vi "Acquire Data.vi"(7 "user event":T2, 8 "error in (no error)":errorcluster, 9 "UI Refs":T1, 10 "Waveforms":waveform(dbl)[](array[waveform]), 11 "XY Plotter":refnum<class "XY Plotter.lvclass">) -> (0 "error out":errorcluster, 3 "XY Plotter out":refnum<class "XY Plotter.lvclass">)   [LabVIEW 2025, in "XY Plotter.lvlib" / "XY Plotter.lvclass"]
uses:
  XY Plotter.lvclass
  Users/Public/Documents/Sandia National Labs/TSS Plugin/CEF.lvlibp/Node/UserEventRef.ctl
  XY Plotter configuration/XY Plotter configuration.lvclass
  XY Plotter configuration/XY Plotter configuration.lvclass/XY Plotter configuration.ctl
  41d9ed76-e5e6-4aa3-be95-e74946f1bf3d.vi
  XY Plotter configuration/Read XY Plotter.vi
  Users/Public/Documents/Sandia National Labs/TSS Plugin/CEF.lvlibp/serializable configuration/CEF_serializable configuration.lvclass
  Users/Public/Documents/Sandia National Labs/TSS Plugin/CEF.lvlibp/Node/CEF_Node.lvclass
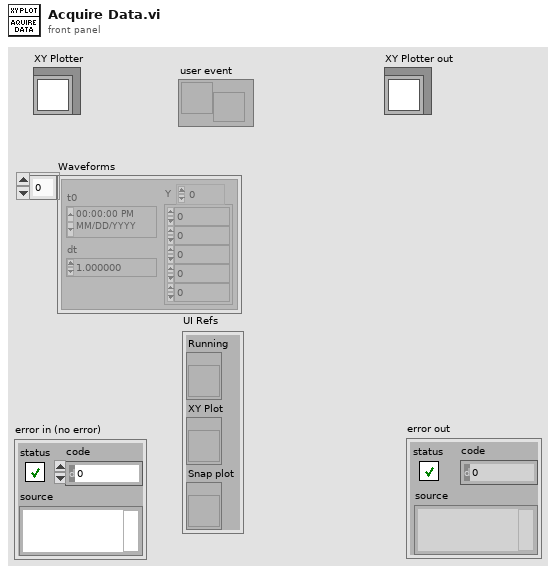
[diagram p1: front panel]
types:
  T1 = cluster{"Running":refnum<vi>, "XY Plot":refnum<vi>, "Snap plot":refnum<vi>}
  T2 = typedef "CEF.lvlibp/CEF_Node.lvclass/UserEventRef.ctl" = refnum<user-event>
  T3 = enum16{"Start Timer", "Read Time", "Pause", "Resume"}
  T4 = typedef "XY Plotter.lvlib/XY Plotter configuration.lvclass/XY Plotter.ctl" = cluster{"Data Rate":i32, "Y-Scales":cluster{"Label":string, "Max":dbl, "Min":dbl, "Unit":enum16{"---", "V", "mA", "sec", "dB", "deg", "in/s", "in", "lbf", "Hz", "psi", "gpm"}, "Visible":bool}[], "Note":string, "History Length":i32, "DataLog Path":path, "Plot type":bool, "X-Scales":cluster{"Label":string, "Max":dbl, "Min":dbl, "Unit":enum16{"---", "V", "mA", "sec", "dB", "deg", "in/s", "in", "lbf", "Hz", "psi", "gpm"}, "Visible":bool}[], "Plot List":cluster{"Plot Name":string, "X Scale Index":u32, "Y Scale Index":u32, "Visible":bool}[]}
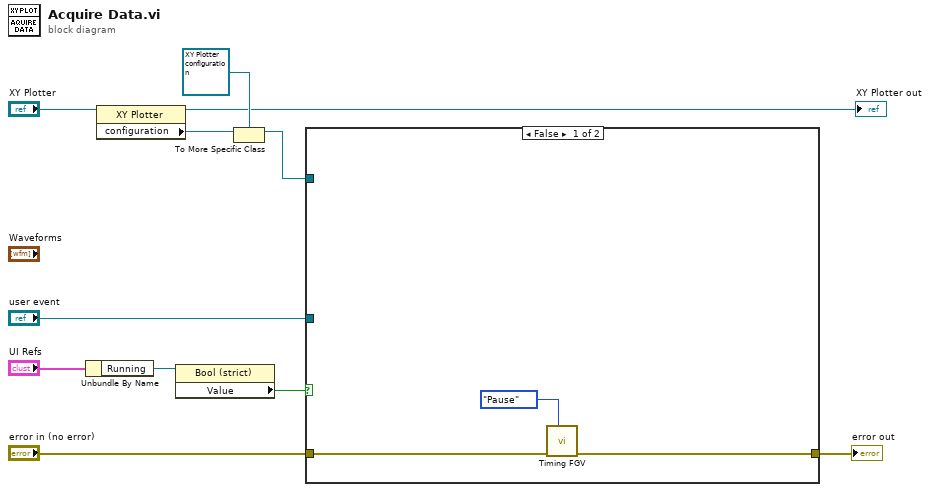
[diagram p0: block diagram]
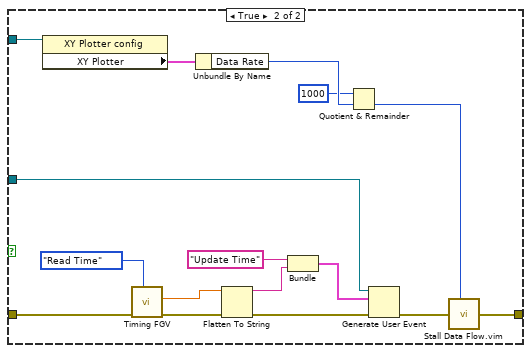
[diagram p2: hidden frame]
diagram:
  n1 = Unbundle By Name("UI Refs") -> ("Running"=w11:refnum<vi>)
  n2 = property class="XY Plotter"(reference="XY Plotter") -> (reference out=→"XY Plotter out":refnum<class "XY Plotter.lvclass">, "configuration"=w8:refnum<class "CEF_serializable configuration.lvclass">)  [unwired: 1 in, 1 out]
  n3 = property class="Bool (strict)"(reference=w11) -> ("Value"=w6:bool)  [unwired: 1 in, 2 out]
  n4 = To More Specific Class(target class=refnum<class "XY Plotter configuration.lvclass"> refnum ("XY Plotter.lvlib:XY Plotter config"), reference=w8) -> (specific class reference=w2:refnum<class "XY Plotter configuration.lvclass">)  [unwired: 1 in, 1 out]
  n5 = case shown="False" w6 {
    tunnel: "user event" -> [_ w22]
    tunnel: "error in (no error)" -> [w14 w30]
    tunnel: [w13 w20] -> w3
    tunnel: w2 -> [_ w18]
    frame False {
      n6 = call "Timing FGV.vi"("Timer Mode"=T3."Pause", "Error In"=w14) -> ("Error Out"=w13:errorcluster)  [unwired: 7 in, 2 out]
    }
    frame True {
      n7 = property class="XY Plotter config"(reference=w18) -> ("XY Plotter"=w19:T4)  [unwired: 1 in, 2 out]
      n8 = call "Timing FGV.vi"("Timer Mode"=T3."Read Time", "Error In"=w30) -> ("Error Out"=w24:errorcluster, "Elapsed Time (s.ms)"=w23:dbl)  [unwired: 7 in, 1 out]
      n9 = Unbundle By Name(w19) -> ("Data Rate"=w17:i32)
      n10 = Flatten To String(anything=w23, error in (no error)=w24) -> (data string=w27:string, error out=w28:errorcluster)  [unwired: 2 in, 1 out]
      n11 = Bundle("message"="Update Time", "data string"=w27) -> (w26:cluster{"message":string, "data string":string})  [unwired: 1 in]
      n12 = Quotient & Remainder(x=1000, y=w17) -> (floor(x/y)=w15:i32)  [unwired: 1 out]
      n13 = Generate User Event(user event=w22, event data cluster=w26, error in=w28) -> (error out=w21:errorcluster)  [unwired: 1 in, 1 out]
      n14 = call "Stall Data Flow.vim"("value in"=w21, "milliseconds to wait"=w15) -> ("value out"=w20:errorcluster)  [unwired: 1 out]
    }
  }
  "error out" <- w3
